vi "Cleanup.vi"(8 "error in (no error)":errorcluster, 11 "App Watcher in":refnum<class "App Watcher.lvclass">) -> (0 "error out":errorcluster)   [LabVIEW 2020, in "PicoG-App.lvlib" / "App Watcher.lvclass"]
uses:
  App Watcher.lvclass
  App Watcher.lvclass/App Watcher.ctl
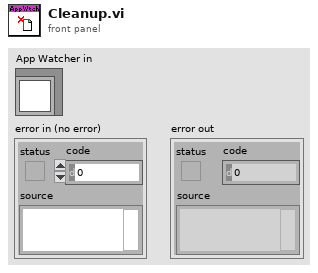
[diagram p1: front panel]
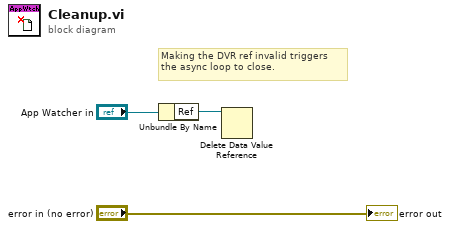
[diagram p0: block diagram]
diagram:
  # "Making the DVR ref invalid triggers the async loop to close."
  n1 = Unbundle By Name("App Watcher in") -> ("Ref"=w1:refnum<data-value>)
  n2 = Delete Data Value Reference(data value reference=w1) -> ()  [unwired: 1 in, 2 out]
  "error out" <- "error in (no error)"
